vi "GetConfigurationType.vi"(8 "error in (no error)":errorcluster, 11 "object in":refnum<class "DIO_Channel.lvclass">) -> (0 "error out":errorcluster, 2 "Configuration":refnum<class "Configuration.lvclass">, 3 "object out":refnum<class "DIO_Channel.lvclass">)   [LabVIEW 2021, in "DIO-Channel.lvlib" / "DIO_Channel.lvclass"]
doc: "Gets the Configuration to use"
uses:
  DIO_Channel.lvclass
  Dependencies/Channel.lvlibp/Channel/Configuration_class/Configuration.lvclass
  DIO-Configuration_class/DIO-Configuration.lvclass
  C:/Users/averna/Documents/LV Gym DEMO/Factory Pattern/Channels/Dependencies/Channel.lvlibp/Channel/Configuration_class/Configuration.lvclass
  DIO_Channel.lvclass/DIO_Channel.ctl
  C:/Users/averna/Documents/LV Gym DEMO/Factory Pattern/Channels/DIO-Channel/DIO-Configuration_class/DIO-Configuration.lvclass
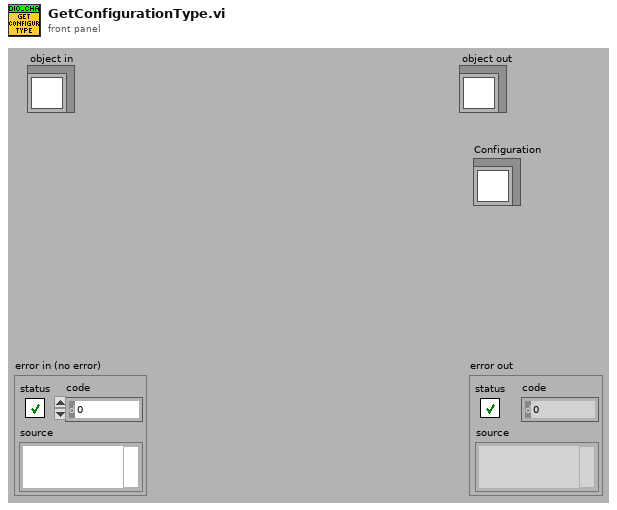
[diagram p1: front panel]
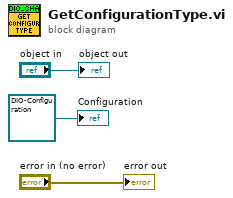
[diagram p0: block diagram]
diagram:
  "error out" <- "error in (no error)"
  "object out" <- "object in"
  "Configuration" <- refnum<class "DIO-Configuration.lvclass"> refnum ("DIO-Channel.lvlib:DIO_CFG")
